vi "Add Error Core.vi"(8 "error in (no error)":errorcluster, 10 "String to Append":string, 11 "Error":T1) -> (0 "error out":errorcluster)   [LabVIEW 2021, in "Iceoryx.lvlib"]
doc: "This reentrant VI contains the error messages. It is called by a wrapper that is inlined for optimal performance. This VI is not inlined to minimize memory impact."
uses:
  Iceoryx.lvlib
  typedef/Errors.ctl
  <vilib>/CIF Foundation/CIF Utilities/Errors/Errors_CIF_U.lvlib
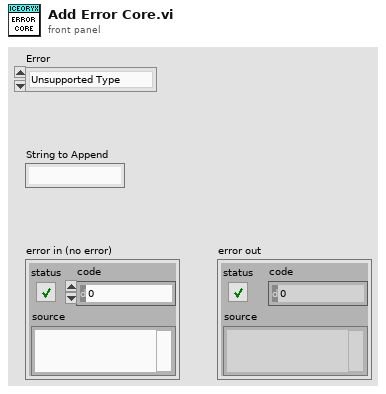
[diagram p1: front panel]
types:
  T1 = typedef "Iceoryx.lvlib/Errors.ctl" = enum16{"Unsupported Type", "Empty Name", "Cluster Name"}
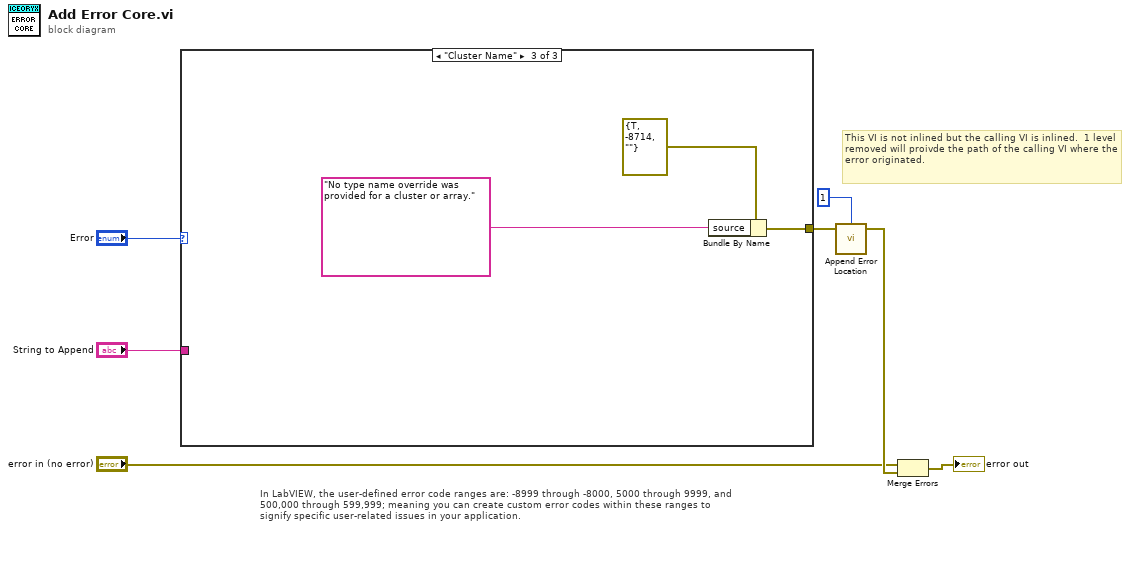
[diagram p0: block diagram]
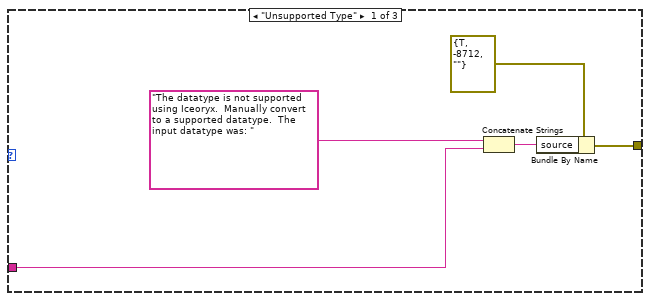
[diagram p2: hidden frame]
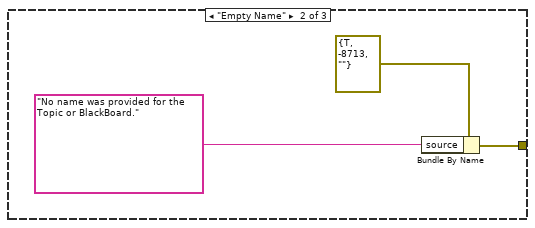
[diagram p3: hidden frame]
diagram:
  # "This VI is not inlined but the calling VI is inlined.  1 level removed will proivde the path of the calling VI where the error originated."
  # "In LabVIEW, the user-defined error code ranges are: -8999 through -8000, 5000 through 9999, and 500,000 through 599,999; meaning you can create custom error codes within these ranges to signify specific user-related issues in your application."
  n1 = case shown="\"Cluster Name\"" "Error" {
    tunnel: "String to Append" -> [w9 _ _]
    tunnel: [w11 w14 w17] -> w6
    frame "Unsupported Type" {
      n2 = Concatenate Strings("The datatype is not supported using Iceoryx.  Manually convert to a supported datatype.  The input datatype was: " ("source"), w9) -> (w8:string)
      n3 = Bundle By Name(cluster=errorcluster {"status"=TRUE, "code"=-8712, "source"=""} ("Invalid ID"), "source"=w8) -> (w11:errorcluster)
    }
    frame "Empty Name" {
      n4 = Bundle By Name(cluster=errorcluster {"status"=TRUE, "code"=-8713, "source"=""} ("Invalid ID"), "source"="No name was provided for the Topic or BlackBoard.") -> (w14:errorcluster)
    }
    frame "Cluster Name" {
      n5 = Bundle By Name(cluster=errorcluster {"status"=TRUE, "code"=-8714, "source"=""} ("Invalid ID"), "source"="No type name override was provided for a cluster or array.") -> (w17:errorcluster)
    }
  }
  n6 = call <vilib>:"Append Error Location.vi"("error in (no error)"=w6, "Chain Depth"=1) -> ("error out"=w7:errorcluster)  [unwired: 3 in]
  n7 = Merge Errors("error in (no error)", w7) -> (→"error out":errorcluster)
